vi "MotorController.vi"   [LabVIEW 2026]
uses:
  <vilib>/DAQmx/write.llb/DAQmx Write (Analog 1D Wfm NChan NSamp).vi
  <vilib>/DAQmx/write.llb/DAQmx Write (Digital Bool 1Line 1Point).vi
  <vilib>/DAQmx/write.llb/DAQmx Write (Analog 2D DBL NChan NSamp).vi
  <vilib>/DAQmx/create/channels.llb/DAQmx Create Channel (DO-Digital Output).vi
  <vilib>/DAQmx/create/channels.llb/DAQmx Create Channel (AO-Voltage-Basic).vi
  <vilib>/DAQmx/configure/timing.llb/DAQmx Timing (Sample Clock).vi
  <vilib>/DAQmx/miscellaneous.llb/DAQmx Fill In Error Info.vi
  StateMachine/Globals.vi
types:
  T1 = typedef "BeltCtrl.ctl" = enum16{"Off", "Forward", "Back", "Coast", "Brake", ""}
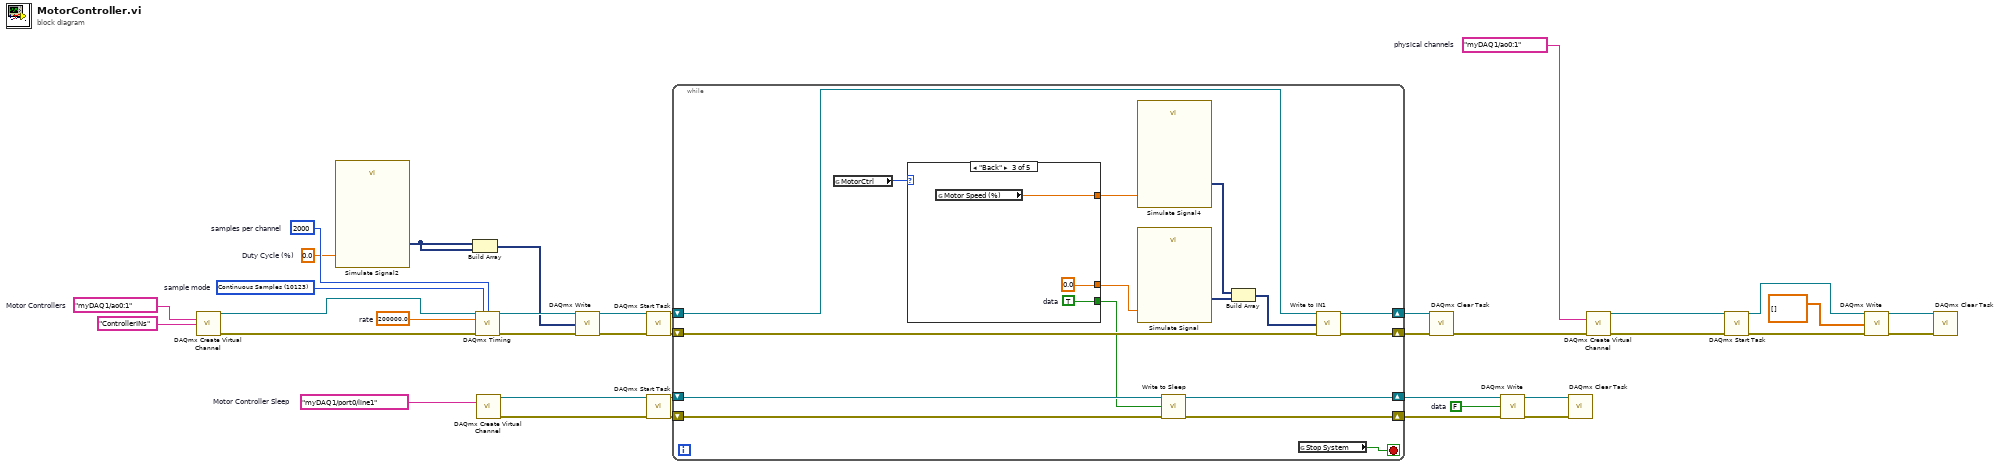
[diagram p0: block diagram]
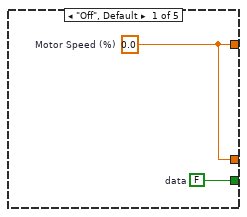
[diagram p2: hidden frame]
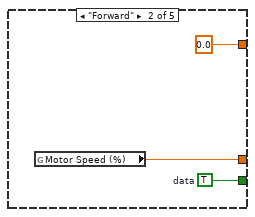
[diagram p3: hidden frame]
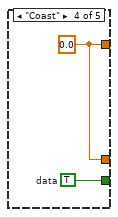
[diagram p4: hidden frame]
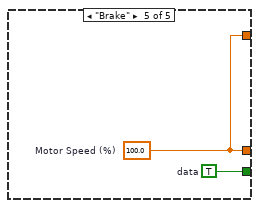
[diagram p5: hidden frame]
diagram:
  w23 = FALSE  # data
  w24 = tag "myDAQ1/port0/line1"  # Motor Controller Sleep
  w25 = 0.0  # Duty Cycle (%)
  w30 = tag "myDAQ1/ao0:1"  # physical channels
  w32 = 2000  # samples per channel
  w33 = 10123 items=["Finite Samples"=10178, "Continuous Samples"=10123, "Hardware Timed Single Point"=12522]  # sample mode
  w34 = 200000.0  # rate
  w37 = tag "myDAQ1/ao0:1"  # Motor Controllers
  n1 = call-poly <vilib>:"DAQmx Create Virtual Channel.vi"("physical channels"=w37, "name to assign"="ControllerINs") -> ("task out"=w36:refnum<k21>, "error out"=w35:errorcluster)  [unwired: 12 in]
  n2 = call "Simulate Signal2"("Duty Cycle (%)"=w25) -> ("Square"=w9:dynamicdata)  [unwired: 13 in, 1 out]
  n3 = Build Array(w9, w9) -> (w8:dynamicdata[])
  n4 = call-poly <vilib>:"DAQmx Timing.vi"("task/channels in"=w36, "sample mode"=w33, "samples per channel"=w32, "rate"=w34, "error in"=w35) -> ("task out"=w29:refnum<k21>, "error out"=w28:errorcluster)  [unwired: 9 in]
  n5 = call-poly <vilib>:"DAQmx Create Virtual Channel.vi"("lines"=w24) -> ("task out"=w20:refnum<k21>, "error out"=w19:errorcluster)  [unwired: 13 in]
  n6 = call-poly <vilib>:"DAQmx Write.vi"("task/channels in"=w29, "data"=w8, "error in"=w28) -> ("task out"=w27:refnum<k21>, "error out"=w26:errorcluster)  [unwired: 10 in, 1 out]
  n7 = call <vilib>:"DAQmx Start Task.vi"("task/channels in"=w27, "error in"=w26) -> ("task out"=w18:refnum<k21>, "error out"=w17:errorcluster)  [unwired: 12 in]
  n8 = call <vilib>:"DAQmx Start Task.vi"("task/channels in"=w20, "error in"=w19) -> ("task out"=w14:refnum<k21>, "error out"=w13:errorcluster)  [unwired: 12 in]
  n9 = while {
    shift-right: [w50] -> w16
    shift-left: w18 -> [w52]
    shift-right: [w49] -> w15
    shift-left: w17 -> [w51]
    shift-right: [w46] -> w12
    shift-left: w14 -> [w48]
    shift-right: [w45] -> w11
    shift-left: w13 -> [w47]
    stop <- w53 stop-if-true
    n10 = global read "Globals.vi" "MotorCtrl"() -> (w44:T1)
    n11 = case shown="\"Back\"" w44 {
      tunnel: [w54 0.0 w60 w62 w65] -> w43
      tunnel: [w55 w57 w59 w63 w64] -> w42
      tunnel: [w54 w56 0.0 w62 w65] -> w41
      frame "Off", Default {
        w54 = 0.0  # Motor Speed (%)
        w55 = FALSE  # data
      }
      frame "Forward" {
        w57 = TRUE  # data
        n12 = global read "Globals.vi" "Motor Speed (%)"() -> (w56:dbl)
      }
      frame "Back" {
        w59 = TRUE  # data
        n13 = global read "Globals.vi" "Motor Speed (%)"() -> (w60:dbl)
      }
      frame "Coast" {
        w63 = TRUE  # data
        w62 = 0.0
      }
      frame "Brake" {
        w64 = TRUE  # data
        w65 = 100.0  # Motor Speed (%)
      }
    }
    n14 = call "Simulate Signal4"("Duty Cycle (%)"=w43) -> ("Square"=w40:dynamicdata)  [unwired: 13 in, 1 out]
    n15 = call "Simulate Signal"("Duty Cycle (%)"=w41) -> ("Square"=w39:dynamicdata)  [unwired: 13 in, 1 out]
    n16 = call-poly "Write to Sleep"("task/channels in"=w48, "data"=w42, "error in"=w47) -> ("task out"=w46:refnum<k21>, "error out"=w45:errorcluster)  [unwired: 10 in, 1 out]
    n17 = Build Array(w40, w39) -> (w38:dynamicdata[])
    n18 = global read "Globals.vi" "Stop System"() -> (w53:bool)
    n19 = call-poly "Write to IN1"("task/channels in"=w52, "data"=w38, "error in"=w51) -> ("task out"=w50:refnum<k21>, "error out"=w49:errorcluster)  [unwired: 10 in, 1 out]
  }
  n20 = call <vilib>:"DAQmx Clear Task.vi"("task in"=w16, "error in"=w15) -> ("error out"=w31:errorcluster)  [unwired: 13 in]
  n21 = call-poly <vilib>:"DAQmx Write.vi"("task/channels in"=w12, "data"=w23, "error in"=w11) -> ("task out"=w22:refnum<k21>, "error out"=w21:errorcluster)  [unwired: 10 in, 1 out]
  n22 = call <vilib>:"DAQmx Clear Task.vi"("task in"=w22, "error in"=w21) -> ()  [unwired: 13 in, 1 out]
  n23 = call-poly <vilib>:"DAQmx Create Virtual Channel.vi"("physical channels"=w30, "error in"=w31) -> ("task out"=w7:refnum<k21>, "error out"=w5:errorcluster)  [unwired: 12 in]
  n24 = call <vilib>:"DAQmx Start Task.vi"("task/channels in"=w7, "error in"=w5) -> ("task out"=w6:refnum<k21>, "error out"=w4:errorcluster)  [unwired: 12 in]
  n25 = call-poly <vilib>:"DAQmx Write.vi"("task/channels in"=w6, "data"=dbl[][] [], "error in"=w4) -> ("task out"=w2:refnum<k21>, "error out"=w1:errorcluster)  [unwired: 10 in, 1 out]
  n26 = call <vilib>:"DAQmx Clear Task.vi"("task in"=w2, "error in"=w1) -> ()  [unwired: 13 in, 1 out]
